vi "VIH Project Tree - Item Type to Boolean Flags (extra #1).vi"(11 "Item Type":T1) -> (2 "Can be documented":bool, 3 "Can have Qualified name":bool)   [LabVIEW 2014]
doc: "::: VI Helpeks :::\nCopyright (c) 2000-2026 Konstantin Shifershteyn. All rights reserved."
uses:
  VIH Project Tree Typedef - Tree Item Type.ctl
panel:
  # "VI Helpeks\nCopyright (c) 2012-2026 Konstantin Shifershteyn"
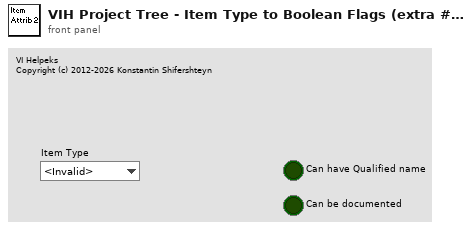
[diagram p1: front panel]
types:
  T1 = typedef "VIH Project Tree Typedef - Tree Item Type.ctl" = enum32{"<Invalid>", "Project", "Proj Files", "Proj Rules", "File Group", "Rule Group", "Any File", "LV Func", ".mnu", ".mnu (dyn)", ".vi", ".vi (dyn)", ".vit", ".vit (dyn)", ".ctl", ".ctl (dyn)", ".ctt", ".ctt (dyn)", "polyVI", "polyVI (dyn)", "expVI", "expVI (dyn)", "HTML", "PolyVI Inst"}
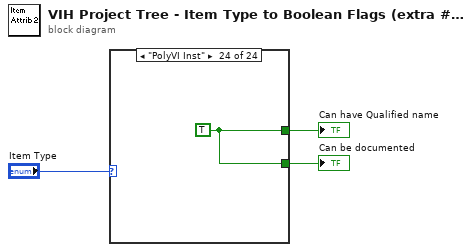
[diagram p0: block diagram]
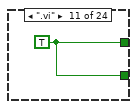
[diagram p12: hidden frame]
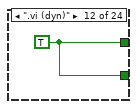
[diagram p13: hidden frame]
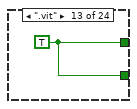
[diagram p14: hidden frame]
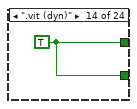
[diagram p15: hidden frame]
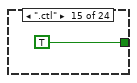
[diagram p16: hidden frame]
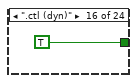
[diagram p17: hidden frame]
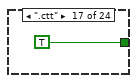
[diagram p18: hidden frame]
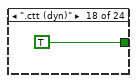
[diagram p19: hidden frame]
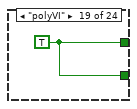
[diagram p20: hidden frame]
diagram:
  n1 = case shown="\"PolyVI Inst\"" "Item Type" {
    tunnel: [_ _ _ _ _ _ _ _ _ _ w4 w5 w6 w7 TRUE TRUE TRUE TRUE w12 w13 TRUE TRUE _ w16] -> w2
    tunnel: [_ _ _ _ _ _ _ _ _ _ w4 w5 w6 w7 _ _ _ _ w12 w13 _ _ _ w16] -> w1
    frame "<Invalid>" {
    }
    frame "Project" {
    }
    frame "Proj Files" {
    }
    frame "Proj Rules" {
    }
    frame "File Group" {
    }
    frame "Rule Group" {
    }
    frame "Any File" {
    }
    frame "LV Func" {
    }
    frame ".mnu" {
    }
    frame ".mnu (dyn)" {
    }
    frame ".vi" {
      w4 = TRUE
    }
    frame ".vi (dyn)" {
      w5 = TRUE
    }
    frame ".vit" {
      w6 = TRUE
    }
    frame ".vit (dyn)" {
      w7 = TRUE
    }
    frame ".ctl" {
    }
    frame ".ctl (dyn)" {
    }
    frame ".ctt" {
    }
    frame ".ctt (dyn)" {
    }
    frame "polyVI" {
      w12 = TRUE
    }
    frame "polyVI (dyn)" {
      w13 = TRUE
    }
    frame "expVI" {
    }
    frame "expVI (dyn)" {
    }
    frame "HTML" {
    }
    frame "PolyVI Inst" {
      w16 = TRUE
    }
  }
  "Can have Qualified name" <- w2
  "Can be documented" <- w1
